vi "Objective Align.vi"(7 "Calling VI Ref":refnum<vi>) -> ()   [LabVIEW 2021]
uses:
  Objective Align Controls/Objective Align Notifier Type Def.ctl
  Objective Align Controls/Objective Align Actions.ctl
  <vilib>/vision/Image Controls.llb/IMAQ Image.ctl
  <vilib>/Utility/miscctls.llb/LVPointTypeDef.ctl
  Hardware Configuration/Hardware Configuration Controls/Device Type.ctl
  Hardware Configuration/Hardware Configuration Controls/Device Function.ctl
  Device Library/Stages/Stages Controls/Stage Actions.ctl
panel:
  in  "Align z":bool
  out "zmoved":bool
  out "Top Z shift":dbl
  out "Bottom Z shift":dbl
  in  "Sample Z factor":dbl=0.55
  in  "Obj. Z factor":dbl=0.55
  in  "Quit":bool
  in  "Frame Accumulation":u16
  in  "CCD offset":dbl
  out "XY shift":dbl[](array[numeric])
  out "Coord":i32[][](array[numeric])
  out "Z metric (top, bottom)":dbl[](array[numeric])
  out "ROI stack":u16[][][](array[numeric])
  in  "ROI Size":i32
  in  "XY Step Size (µm)":dbl
  in  "Pixel Size (µm)":dbl
  in  "Start Align":bool
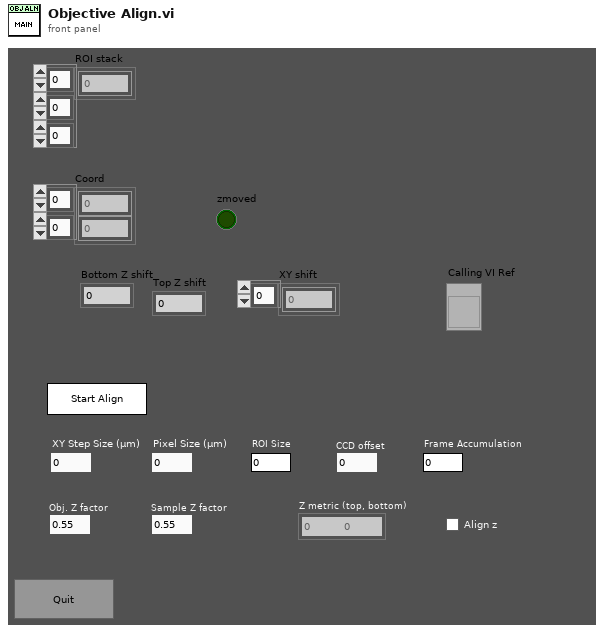
[diagram p1: front panel]
types:
  T1 = enum16{"Always On", "Always Off", "Off While Running"}
  T2 = typedef "LVPointTypeDef.ctl" = cluster{"Horizontal":i16, "Vertical":i16}
  T3 = typedef "IMAQ Image.ctl" = refnum<image>
  T4 = typedef "Objective Align Actions.ctl" = enum16{"idle", "Start Align", "Move Z stage", "Move XY Stage", "Get Image", "Get Position", "Exit", "Quit"}
  T5 = typedef "Objective Align Notifier Type Def.ctl" = cluster{"Action":T4, "Pixel Size (µm)":dbl, "XY Step Size (µm)":dbl, "Image Ref":T3, "ROI Size":i32, "ROI Stack":u16[][][], "Frame Accumulation":u16, "CCD offset":dbl, "obj. Z factor":dbl, "sample Z factor ":dbl}
  T6 = typedef "Device Function.ctl" = enum16{"Primary", "Secondary", "Overview", "Wide Field Drift Correction", "642 nm Excitation", "560 nm Excitation", "940 nm Excitation", "546 nm Excitation", "488 nm Excitation", "405 nm Excitation", "Objective Drift Correction", "4Pi Focus Lock", "4Pi Objective Lock", "Objective XY", "Objective Z", "Sample XY", "Sample Coarse Z", "Sample Z", "4Pi Lower", "4Pi Upper", "Em Small", "Em Large", "Ex Small", "Ex Large", "Mojo", "Adj Cavity", "Line Scanning", "Alert"}
  T7 = typedef "Device Type.ctl" = enum16{"AOTF", "Camera", "Deformable Mirror", "Laser", "Flip Mirror", "Shutter", "Stage", "Waveform", "FPGA", "Filter Wheel", "Email"}
  T8 = typedef "Stage Actions.ctl" = enum16{"Get Position", "SERVO OFF", "SERVO ON", "SERVO ON/OFF", "MVR", "MOVE", "HALT", "ONTARGET", "ERROR", "REFERENCE", "INIT", "VELOCITY", "STATUS", "EXIT", "HOME", "ZEROPOS", "NANOPOS", "ANALOG", "QUIT"}
  T9 = typedef "4Pi OBJ Lock-2D Gaussian - Best Fit Parameters.ctl" = cluster{"Amplitude":dbl, "X Position":dbl, "Y Position":dbl, "X Width":dbl, "Y Width":dbl, "Offset":dbl}
  T10 = typedef "LVRectTypeDef.ctl" = cluster{"Left":i16, "Top":i16, "Right":i16, "Bottom":i16}
  T11 = typedef "LVBoundsTypeDef.ctl" = cluster{"Width":u32, "Height":u32}
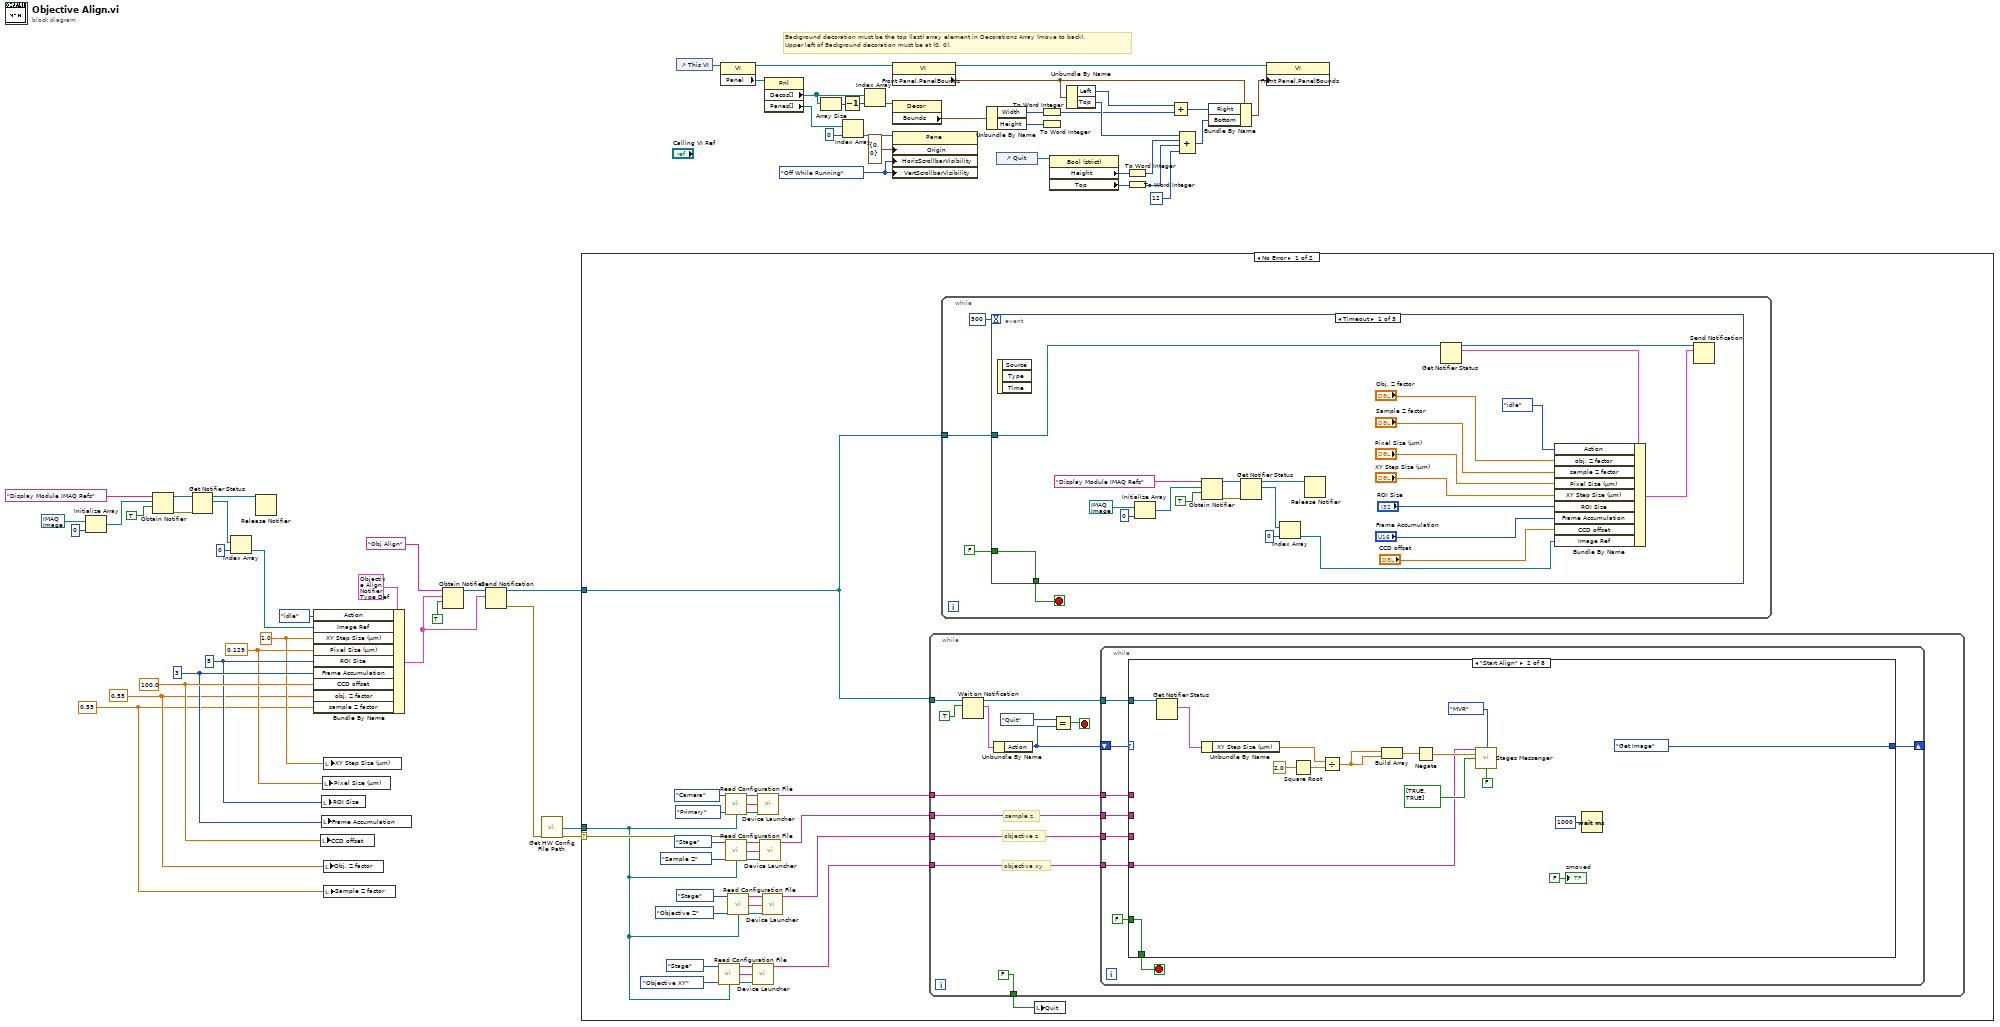
[diagram p0: block diagram]
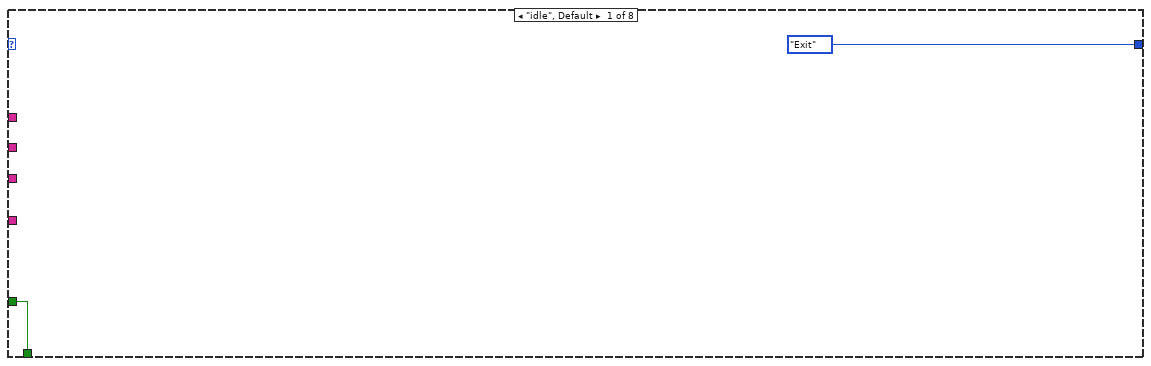
[diagram p2: hidden frame]
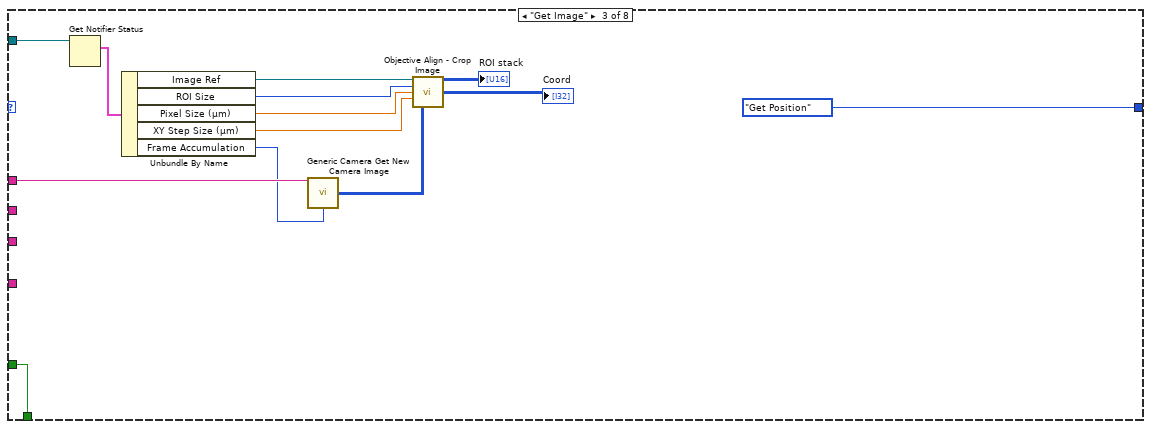
[diagram p3: hidden frame]
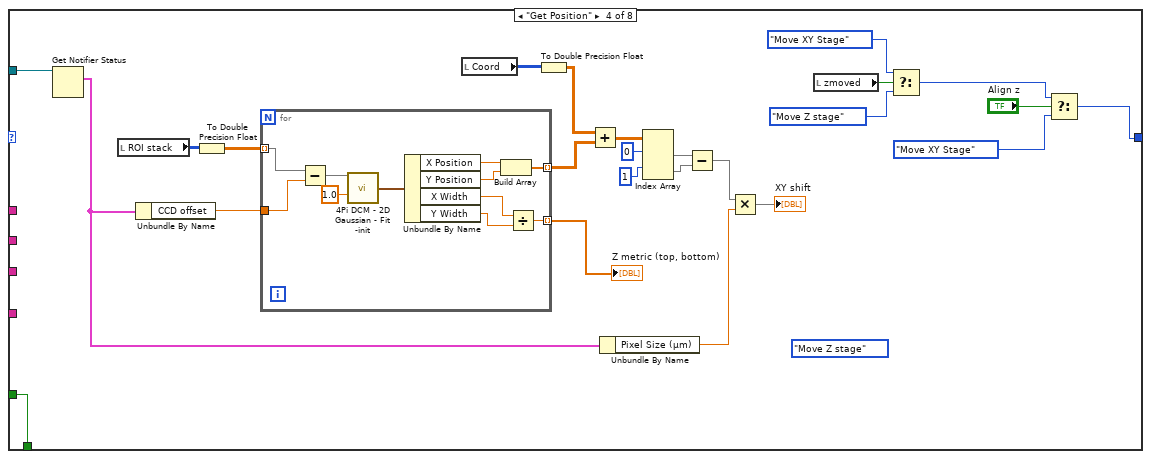
[diagram p4: hidden frame]
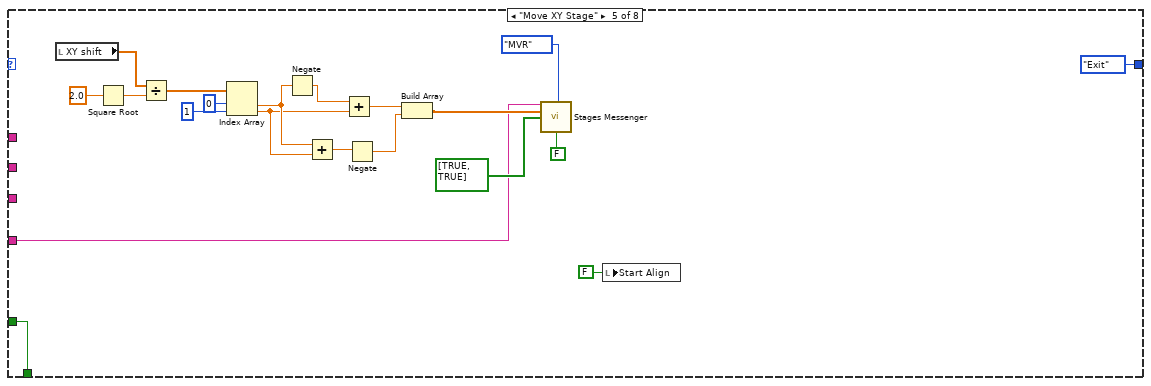
[diagram p5: hidden frame]
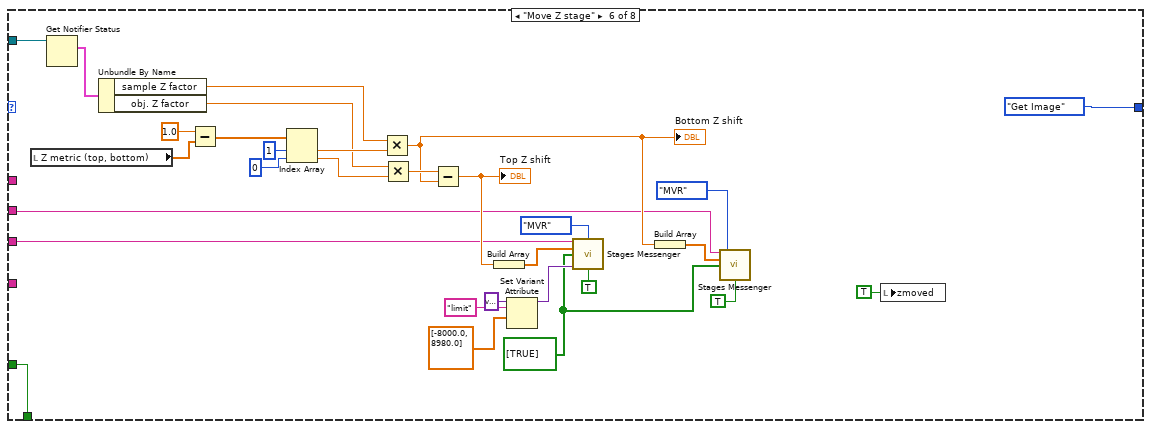
[diagram p6: hidden frame]
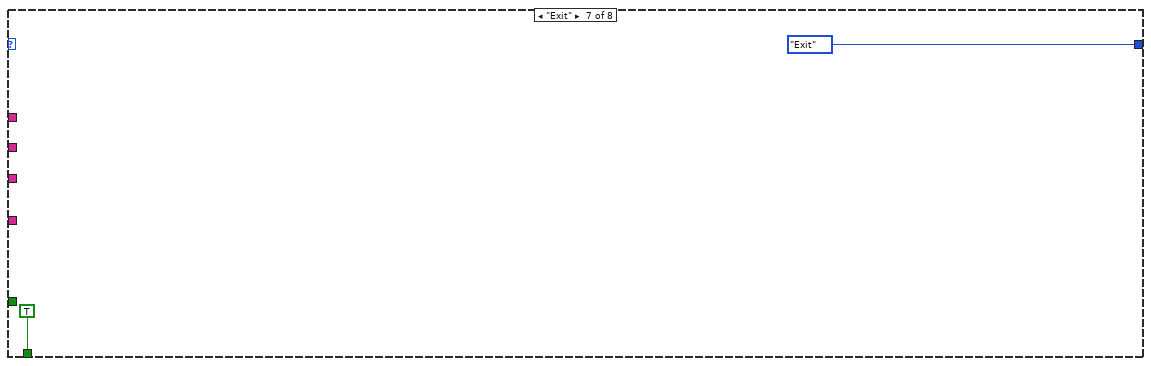
[diagram p7: hidden frame]
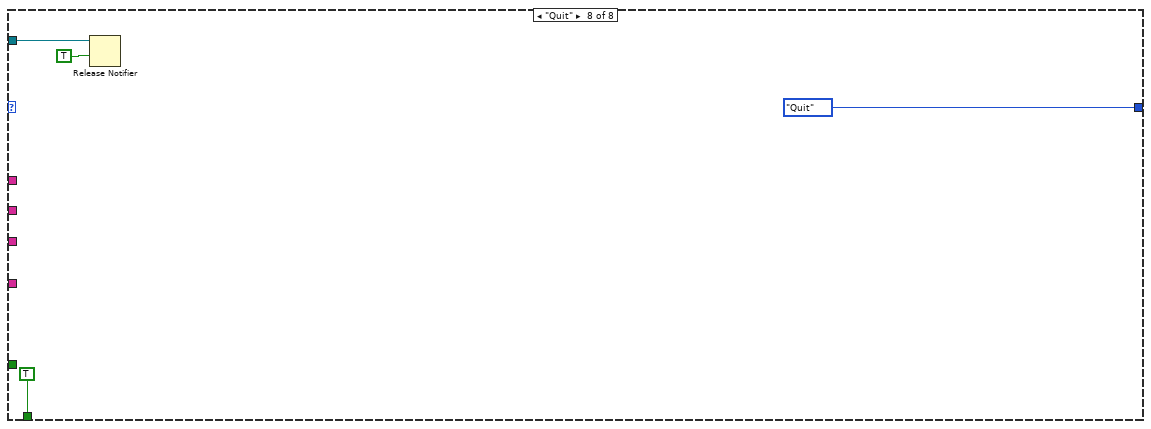
[diagram p8: hidden frame]
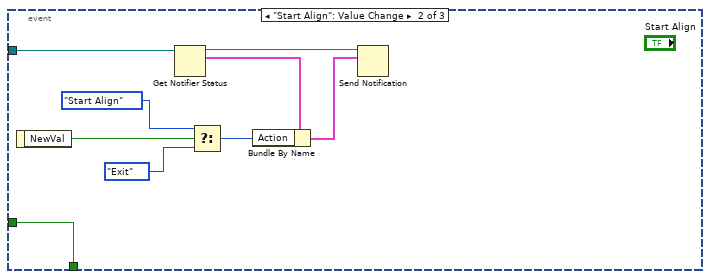
[diagram p9: hidden frame]
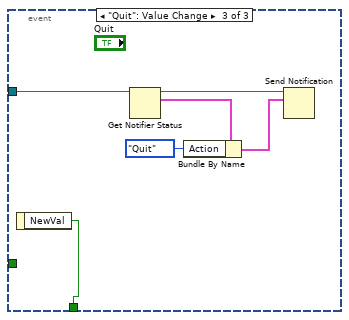
[diagram p10: hidden frame]
diagram:
  w1 = 0.55 ("sample Z factor")
  w2 = 0.55 ("obj. Z factor")
  w15 = T1."Off While Running" ("Vertical Scrollbar Visibility")
  w38 = 100.0 ("CCD offset")
  w37 = u16 3 ("Frame Accumulation")
  w36 = 5 ("ROI Size")
  w35 = 0.129 ("Pixel Size (µm)")
  w34 = 1.0 ("XY Step Size (µm)")
  # "Background decoration must be the top (last) array element in Decorations Array (move to back).\nUpper left of Background decoration must be at (0, 0)."
  n1 = Initialize Array(T3 refnum ("New Image"), 0 ("dimension size")) -> (w51:T3[])
  n2 = Obtain Notifier(name (unnamed)="Display Module IMAQ Refs", notification data type=w51, create if not found? (T)=TRUE) -> (notifier out=w50:refnum<notifier>, error out=w49:errorcluster)  [unwired: 1 in, 1 out]
  n3 = Get Notifier Status(notifier=w50, error in (no error)=w49) -> (notifier out=w3:refnum<notifier>, current notification=w48:T3[])  [unwired: 3 out]
  n4 = Index Array(array=w48, index=0) -> (element=w46:T3)
  n5 = Release Notifier(notifier=w3) -> ()  [unwired: 2 in, 3 out]
  n6 = Bundle By Name(cluster=T5 {"Action"=enum."Start Align", "Pixel Size (µm)"=0.0, "XY Step Size (µm)"=0.0, "Image Ref"=refnum, "ROI Size"=0, "ROI Stack"=[], "Frame Accumulation"=0, "CCD offset"=0.0, "obj. Z factor"=0.0, "sample Z factor "=0.0} ("Objective Align Notifier Type"), "Action"=Objective_Align_Actions."idle", "Image Ref"=w46, "XY Step Size (µm)"=w34, "Pixel Size (µm)"=w35, "ROI Size"=w36, "Frame Accumulation"=w37, "CCD offset"=w38, "obj. Z factor"=w2, "sample Z factor"=w1) -> (w43:T5)
  n7 = local write "CCD offset"(w38) -> ()
  n8 = local write "Frame Accumulation"(w37) -> ()
  n9 = local write "ROI Size"(w36) -> ()
  n10 = local write "Pixel Size (µm)"(w35) -> ()
  n11 = local write "Obj. Z factor"(w2) -> ()
  n12 = local write "XY Step Size (µm)"(w34) -> ()
  n13 = local write "Sample Z factor"(w1) -> ()
  n14 = Obtain Notifier(name (unnamed)="Obj Align", notification data type=w43, create if not found? (T)=TRUE) -> (notifier out=w44:refnum<notifier>)  [unwired: 1 in, 2 out]
  n15 = Send Notification(notification=w43, notifier=w44) -> (notifier out=w39:refnum<notifier>, error out=w42:errorcluster)  [unwired: 1 in]
  n16 = call "Get HW Config File Path.vi"("Error"=w42) -> ("File Path"=w40:path, "Error"=w41:errorcluster)  [unwired: 13 in]
  n17 = case shown="No Error" w41 {
    tunnel: w39 -> [w74 _]
    tunnel: w40 -> [w60 _]
    frame No Error {
      n18 = call "Read Configuration File.vi"("Device Type"=Device_Type."Stage", "Device Function"=Device_Function."Objective XY", "Config File Path"=w60) -> ("Unique Notifier Name"=w79:string, "Device Ports/IDs/Channels"=w78:string[], "Device Engine Path"=w77:path)  [unwired: 9 in, 1 out]
      n19 = call "Read Configuration File.vi"("Device Type"=Device_Type."Camera", "Device Function"=Device_Function."Primary", "Config File Path"=w60) -> ("Unique Notifier Name"=w84:string, "Device Ports/IDs/Channels"=w82:string[], "Device Engine Path"=w83:path)  [unwired: 9 in, 1 out]
      n20 = call "Read Configuration File.vi"("Device Type"=Device_Type."Stage", "Device Function"=Device_Function."Sample Z", "Config File Path"=w60) -> ("Unique Notifier Name"=w69:string, "Device Ports/IDs/Channels"=w70:string[], "Device Engine Path"=w71:path)  [unwired: 9 in, 1 out]
      n21 = call "Read Configuration File.vi"("Device Type"=Device_Type."Stage", "Device Function"=Device_Function."Objective Z", "Config File Path"=w60) -> ("Unique Notifier Name"=w61:string, "Device Ports/IDs/Channels"=w62:string[], "Device Engine Path"=w63:path)  [unwired: 9 in, 1 out]
      n22 = call "Device Launcher.vi"("Notifier Name"=w79, "Device Ports/IDs/Channels"=w78, "Device Engine Path"=w77) -> ("Notifier Name"=w73:string)  [unwired: 11 in, 1 out]
      n23 = call "Device Launcher.vi"("Notifier Name"=w84, "Device Ports/IDs/Channels"=w82, "Device Engine Path"=w83) -> ("Notifier Name"=w72:string)  [unwired: 11 in, 1 out]
      n24 = call "Device Launcher.vi"("Notifier Name"=w69, "Device Ports/IDs/Channels"=w70, "Device Engine Path"=w71) -> ("Notifier Name"=w66:string)  [unwired: 11 in, 1 out]
      n25 = call "Device Launcher.vi"("Notifier Name"=w61, "Device Ports/IDs/Channels"=w62, "Device Engine Path"=w63) -> ("Notifier Name"=w59:string)  [unwired: 11 in, 1 out]
      n26 = while {
        tunnel: w74 -> [w94]
        tunnel: w73 -> [w89]
        tunnel: w72 -> [w88]
        tunnel: w66 -> [w87]
        tunnel: w59 -> [w86]
        tunnel: [FALSE ("Quit")] -> w58
        stop <- w92 stop-if-true
        # "objective xy"
        # "sample z"
        # "objective z"
        n27 = Wait on Notification(notifier=w94, ignore previous (F)=TRUE) -> (notifier out=w91:refnum<notifier>, notification=w95:T5)  [unwired: 2 in, 2 out]
        n28 = Unbundle By Name(w95) -> ("Action"=w90:T4)
        n29 = Equal?(x=Objective_Align_Actions."Quit", y=w90) -> (x = y?=w92:bool)
        n30 = while {
          tunnel: w91 -> [w102]
          shift-right: [w100] -> _
          shift-left: w90 -> [w103]
          tunnel: w89 -> [w101]
          tunnel: w88 -> [w99]
          tunnel: w87 -> [w98]
          tunnel: w86 -> [w97]
          stop <- w104 stop-if-true
          n31 = case shown="\"Start Align\"" w103 {
            tunnel: FALSE -> [w106 w123 w124 w161 w175 w221 _ _]
            tunnel: [w106 w123 w124 w161 w175 w221 TRUE TRUE] -> w104
            tunnel: w102 -> [_ w122 w136 w160 _ w220 _ w227]
            tunnel: w101 -> [_ w111 _ _ w176 _ _ _]
            tunnel: [Objective_Align_Actions."Exit" ("Action") Objective_Align_Actions."Get Image" ("Action") Objective_Align_Actions."Get Position" ("Action") w137 Objective_Align_Actions."Exit" ("Action") Objective_Align_Actions."Get Image" ("Action") Objective_Align_Actions."Exit" ("Action") Objective_Align_Actions."Quit" ("Action")] -> w100
            tunnel: w99 -> [_ _ w134 _ _ _ _ _]
            tunnel: w98 -> [_ _ _ _ _ w197 _ _]
            tunnel: w97 -> [_ _ _ _ _ w201 _ _]
            frame "idle", Default {
            }
            frame "Start Align" {
              n32 = Get Notifier Status(notifier=w122) -> (current notification=w121:T5)  [unwired: 1 in, 4 out]
              n33 = Unbundle By Name(w121) -> ("XY Step Size (µm)"=w118:dbl)
              n34 = Square Root(x=2.0) -> (sqrt(x)=w119:dbl)
              n35 = Divide(x=w118, y=w119) -> (x/y=w117:dbl)
              n36 = Build Array(w117, w117) -> (w116:dbl[])
              n37 = Negate(x=w116) -> (-x=w114:dbl[])
              n38 = call "Stages Messenger.vi"("Stage Notifier Name"=w111, "Actions"=Stage_Actions."MVR", "Setpoint"=w114, "Axis"=bool[] [TRUE, TRUE], "Exit While Busy?"=FALSE) -> ()  [unwired: 6 in, 5 out]
              n39 = Wait (ms)(milliseconds to wait=u32 1000) -> ()  [unwired: 1 out]
              "zmoved" <- FALSE ("zmoved")
            }
            frame "Get Image" {
              n40 = Get Notifier Status(notifier=w136) -> (current notification=w135:T5)  [unwired: 1 in, 4 out]
              n41 = Unbundle By Name(w135) -> ("Image Ref"=w132:T3, "ROI Size"=w131:i32, "Pixel Size (µm)"=w130:dbl, "XY Step Size (µm)"=w129:dbl, "Frame Accumulation"=w133:u16)
              n42 = call "Generic Camera Get New Camera Image.vi"("Camera Notifier Name"=w134, "Frames"=w133) -> ("Image - U16"=w128:u16[][])  [unwired: 11 in, 2 out]
              n43 = call "Objective Align - Crop Image.vi"("Image Ref"=w132, "ROI Size"=w131, "Pixel Size (µm)"=w130, "XY Step Size (µm)"=w129, "Input Image - U16"=w128) -> ("Output Image Stack"=→"ROI stack":u16[][][], "Coord"=→"Coord":i32[][])  [unwired: 9 in]
            }
            frame "Get Position" {
              (unwired) Objective_Align_Actions."Move Z stage" ("Action")
              n44 = Get Notifier Status(notifier=w160) -> (current notification=w147:T5)  [unwired: 1 in, 4 out]
              n45 = local read "ROI stack"() -> (w159:u16[][][])
              n46 = Unbundle By Name(w147) -> ("CCD offset"=w157:dbl)
              n47 = To Double Precision Float(number=w159) -> (double precision float=w158:dbl[][][])
              n48 = for {
                tunnel: w158 -> [w170] mode=indexing
                tunnel: w157 -> [w169]
                tunnel: [w165] -> w156 mode=indexing
                tunnel: [w162] -> w153 mode=indexing
                n49 = Subtract(x=w170, y=w169) -> (x-y=w168:dbl[][])
                n50 = call "4Pi DCM - 2D Gaussian - Fit -init.vi"("Image In (DBL)"=w168, "width"=1.0) -> ("Best Fit Params"=w171:T9)  [unwired: 12 in, 1 out]
                n51 = Unbundle By Name(w171) -> ("X Position"=w164:dbl, "Y Position"=w163:dbl, "X Width"=w167:dbl, "Y Width"=w166:dbl)
                n52 = Build Array(w164, w163) -> (w162:dbl[])
                n53 = Divide(x=w167, y=w166) -> (x/y=w165:dbl)
              }
              "Z metric (top, bottom)" <- w156
              n54 = local read "Coord"() -> (w155:i32[][])
              n55 = To Double Precision Float(number=w155) -> (double precision float=w154:dbl[][])
              n56 = Add(x=w154, y=w153) -> (x+y=w150:dbl[][])
              n57 = Unbundle By Name(w147) -> ("Pixel Size (µm)"=w145:dbl)
              n58 = Index Array(array=w150, index (row) #1=0 ("index"), index (row) #2=1 ("index")) -> (element #1=w149:dbl[], element #2=w148:dbl[])  [unwired: 2 in]
              n59 = Subtract(x=w149, y=w148) -> (x-y=w146:dbl[])
              n60 = Multiply(x=w146, y=w145) -> (x*y=→"XY shift":dbl[])
              n61 = local read "zmoved"() -> (w141:bool)
              n62 = Select(t=Objective_Align_Actions."Move XY Stage" ("f"), s=w141, f=Objective_Align_Actions."Move Z stage" ("Action")) -> (s? t:f=w138:T4)
              n63 = Select(t=w138, s="Align z", f=Objective_Align_Actions."Move XY Stage") -> (s? t:f=w137:T4)
            }
            frame "Move XY Stage" {
              n64 = local read "XY shift"() -> (w188:dbl[])
              n65 = Square Root(x=2.0) -> (sqrt(x)=w189:dbl)
              n66 = Divide(x=w188, y=w189) -> (x/y=w187:dbl[])
              n67 = Index Array(array=w187, index #1=0 ("index"), index #2=1 ("index")) -> (element #1=w185:dbl, element #2=w184:dbl)
              n68 = Negate(x=w185) -> (-x=w186:dbl)
              n69 = Add(x=w185, y=w184) -> (x+y=w183:dbl)
              n70 = Add(x=w186, y=w184) -> (x+y=w179:dbl)
              n71 = Negate(x=w183) -> (-x=w178:dbl)
              n72 = Build Array(w179, w178) -> (w177:dbl[])
              n73 = call "Stages Messenger.vi"("Stage Notifier Name"=w176, "Actions"=Stage_Actions."MVR", "Setpoint"=w177, "Axis"=bool[] [TRUE, TRUE], "Exit While Busy?"=FALSE) -> ()  [unwired: 6 in, 5 out]
              n74 = local write "Start Align"(FALSE ("Start Align")) -> ()
            }
            frame "Move Z stage" {
              w196 = bool[] [TRUE]
              n75 = local read "Z metric (top, bottom)"() -> (w215:dbl[])
              n76 = Get Notifier Status(notifier=w220) -> (current notification=w219:T5)  [unwired: 1 in, 4 out]
              n77 = Unbundle By Name(w219) -> ("sample Z factor"=w212:dbl, "obj. Z factor"=w210:dbl)
              n78 = Subtract(x=1.0, y=w215) -> (x-y=w214:dbl[])
              n79 = Index Array(array=w214, index #1=1 ("index"), index #2=0 ("index")) -> (element #1=w213:dbl, element #2=w211:dbl)
              n80 = Multiply(x=w212, y=w213) -> (x*y=w199:dbl)
              "Bottom Z shift" <- w199
              n81 = Multiply(x=w210, y=w211) -> (x*y=w209:dbl)
              n82 = Subtract(x=w209, y=w199) -> (x-y=w208:dbl)
              "Top Z shift" <- w208
              n83 = Build Array(w208) -> (w202:dbl[])
              n84 = Set Variant Attribute(Variant=variant ("variant"), name="limit", value=dbl[] [-8000.0, 8980.0] ("Array")) -> (Variant out=w203:variant)  [unwired: 1 in, 2 out]
              n85 = call "Stages Messenger.vi"("Stage Notifier Name"=w201, "Actions"=Stage_Actions."MVR", "Setpoint"=w202, "Axis"=w196, "Misc"=w203, "Exit While Busy?"=TRUE) -> ()  [unwired: 5 in, 5 out]
              n86 = Build Array(w199) -> (w198:dbl[])
              n87 = call "Stages Messenger.vi"("Stage Notifier Name"=w197, "Actions"=Stage_Actions."MVR", "Setpoint"=w198, "Axis"=w196, "Exit While Busy?"=TRUE) -> ()  [unwired: 6 in, 5 out]
              n88 = local write "zmoved"(TRUE ("zmoved")) -> ()
            }
            frame "Exit" {
            }
            frame "Quit" {
              n89 = Release Notifier(notifier=w227, force destroy? (F)=TRUE) -> ()  [unwired: 1 in, 3 out]
            }
          }
        }
      }
      n90 = while {
        tunnel: w74 -> [w230]
        stop <- w231 stop-if-true
        n91 = event shown="[0] Timeout" {
          selector: _ -> [_ _ _]
          dyn-events: _ -> [_ _ _]
          timeout: 500 -> [_ _ _]
          tunnel: [w256 w257 w271] -> w231
          tunnel: FALSE -> [w256 w257 _]
          tunnel: w230 -> [w255 w262 w267]
          event Timeout {
            n92 = event-data() -> ()  [unwired: 1 in, 3 out]
            n93 = Initialize Array(T3 refnum ("New Image"), 0 ("dimension size")) -> (w242:T3[])
            n94 = Obtain Notifier(name (unnamed)="Display Module IMAQ Refs", notification data type=w242, create if not found? (T)=TRUE) -> (notifier out=w241:refnum<notifier>, error out=w240:errorcluster)  [unwired: 1 in, 1 out]
            n95 = Get Notifier Status(notifier=w241, error in (no error)=w240) -> (notifier out=w237:refnum<notifier>, current notification=w239:T3[])  [unwired: 3 out]
            n96 = Index Array(array=w239, index=0) -> (element=w236:T3)
            n97 = Release Notifier(notifier=w237) -> ()  [unwired: 2 in, 3 out]
            n98 = Get Notifier Status(notifier=w255) -> (notifier out=w247:refnum<notifier>, current notification=w254:T5)  [unwired: 1 in, 3 out]
            n99 = Bundle By Name(cluster=w254, "Action"=Objective_Align_Actions."idle", "obj. Z factor"="Obj. Z factor", "sample Z factor"="Sample Z factor", "Pixel Size (µm)"="Pixel Size (µm)", "XY Step Size (µm)"="XY Step Size (µm)", "ROI Size"="ROI Size", "Frame Accumulation"="Frame Accumulation", "CCD offset"="CCD offset", "Image Ref"=w236) -> (w248:T5)
            n100 = Send Notification(notification=w248, notifier=w247) -> ()  [unwired: 1 in, 2 out]
          }
          event "Start Align": Value Change {
            n101 = event-data() -> ("NewVal"=w261:bool)  [unwired: 1 in]
            n102 = Get Notifier Status(notifier=w262) -> (notifier out=w264:refnum<notifier>, current notification=w265:T5)  [unwired: 1 in, 3 out]
            n103 = Select(t=Objective_Align_Actions."Start Align" ("Action"), s=w261, f=Objective_Align_Actions."Exit") -> (s? t:f=w258:T4)
            n104 = Bundle By Name(cluster=w265, "Action"=w258) -> (w263:T5)
            n105 = Send Notification(notification=w263, notifier=w264) -> ()  [unwired: 1 in, 2 out]
          }
          event "Quit": Value Change {
            n106 = event-data() -> ("NewVal"=w271:bool)  [unwired: 1 in]
            n107 = Get Notifier Status(notifier=w267) -> (notifier out=w270:refnum<notifier>, current notification=w269:T5)  [unwired: 1 in, 3 out]
            n108 = Bundle By Name(cluster=w269, "Action"=Objective_Align_Actions."Quit") -> (w268:T5)
            n109 = Send Notification(notification=w268, notifier=w270) -> ()  [unwired: 1 in, 2 out]
          }
        }
      }
      n110 = local write "Quit"(w58) -> ()
    }
    frame Error {
    }
  }
  n111 = control-ref of="This VI"() -> (w8:refnum<vi>)
  n112 = property class="VI"(reference=w8) -> (reference out=w16:refnum<vi>, "Panel"=w9:refnum<vi>)  [unwired: 1 in, 1 out]
  n113 = property class="Pnl"(reference=w9) -> ("Decos[]"=w7:refnum<vi>[], "Panes[]"=w12:refnum<vi>[])  [unwired: 1 in, 2 out]
  n114 = Array Size(array=w7) -> (size(s)=w5:i32)
  n115 = Decrement(x=w5) -> (x-1=w6:i32)
  n116 = Index Array(array=w12, index=0) -> (element=w11:refnum<vi>)
  n117 = Index Array(array=w7, index=w6) -> (element=w14:refnum<vi>)
  n118 = property class="VI"(reference=w16) -> (reference out=w18:refnum<vi>, "Front Panel.PanelBounds"=w19:T10)  [unwired: 1 in, 1 out]
  n119 = property class="Decor"(reference=w14) -> ("Bounds"=w17:T11)  [unwired: 1 in, 2 out]
  n120 = property class="Pane"(reference=w11, "Origin"=T2 {"Horizontal"=0, "Vertical"=0}, "HorizScrollbarVisibility"=w15, "VertScrollbarVisibility"=w15) -> ()  [unwired: 1 in, 2 out]
  n121 = Unbundle By Name(w17) -> ("Width"=w22:u32, "Height"=w25:u32)
  n122 = control-ref of="Quit"() -> (w4:refnum<vi>)
  n123 = To Word Integer(number=w22) -> (16bit integer=w24:i16)
  n124 = To Word Integer(number=w25) -> ()  [unwired: 1 out]
  n125 = property class="Bool (strict)"(reference=w4) -> ("Height"=w27:u32, "Top"=w28:i32)  [unwired: 1 in, 2 out]
  n126 = Unbundle By Name(w19) -> ("Left"=w21:i16, "Top"=w32:i16)
  n127 = To Word Integer(number=w27) -> (16bit integer=w30:i16)
  n128 = To Word Integer(number=w28) -> (16bit integer=w31:i16)
  n129 = Add(x=w21, y=w24) -> (x+y=w23:i16)
  n130 = Compound Arithmetic op=ADD(w32, w30, w31, i16 12 ("y")) -> (w26:i16)
  n131 = Bundle By Name(cluster=w19, "Right"=w23, "Bottom"=w26) -> (w20:T10)
  n132 = property class="VI"(reference=w18, "Front Panel.PanelBounds"=w20) -> ()  [unwired: 1 in, 2 out]
